vi "Run Storage Tests.vi"(8 "error in (no error)":errorcluster, 11 "Work Folder":path) -> (0 "error out":errorcluster, 2 "Report":string, 3 "All Passed":bool)   [LabVIEW 2026]
doc: "Runs every Storage test VI (Tests\\Storage) and reports one overall result. Test Data Folder is Tests\\Storage\\Test Data next to this VI; each test copies what it needs from there into a new case folder under Work Folder, so the tests can be repeated and never touch the real data in %LOCALAPPDATA%\\LVTimeTracker. An empty Work Folder (or Not a Path) means the system temp folder, in a subfolder named LVTimeTracker Tests.\n\nAll Passed is TRUE only when every test passed; Report holds every check of every test.\n\nGenerated by: Claude"
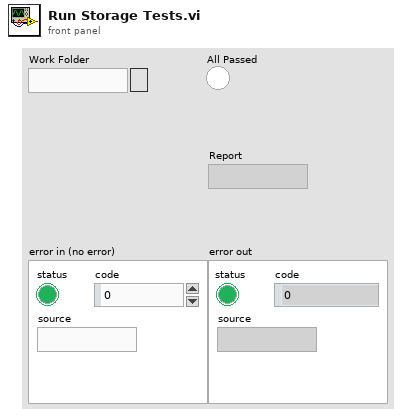
[diagram p1: front panel]
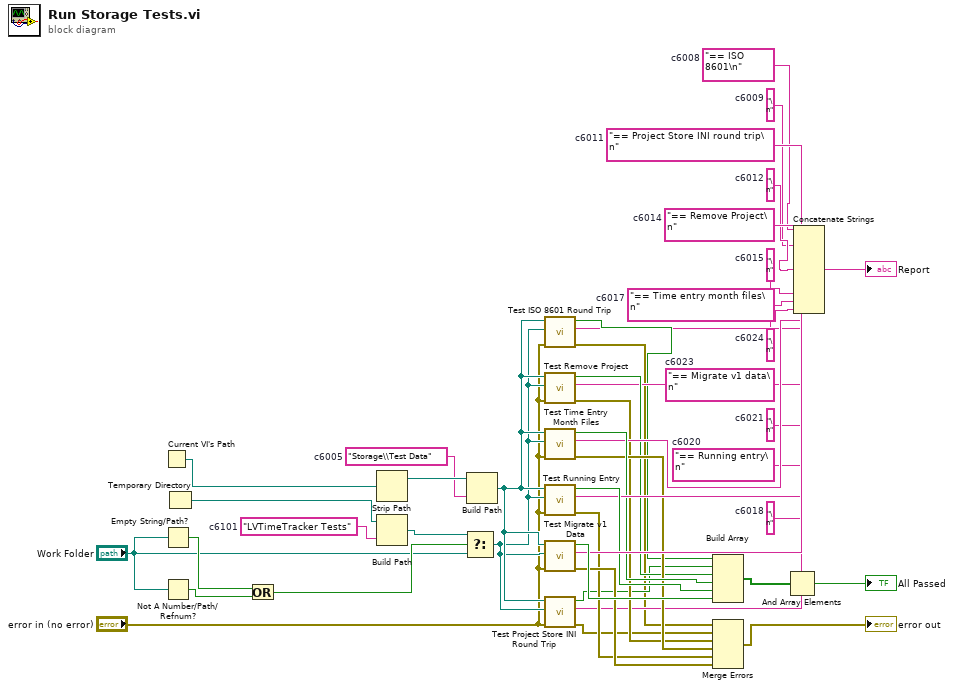
[diagram p0: block diagram]
diagram:
  w20 = "LVTimeTracker Tests"  # c6101
  w18 = "\n"  # c6024
  w17 = "== Migrate v1 data\n"  # c6023
  w16 = "\n"  # c6021
  w15 = "== Running entry\n"  # c6020
  w14 = "\n"  # c6018
  w13 = "== Time entry month files\n"  # c6017
  w12 = "\n"  # c6015
  w11 = "== Remove Project\n"  # c6014
  w10 = "\n"  # c6012
  w9 = "== Project Store INI round trip\n"  # c6011
  w8 = "\n"  # c6009
  w7 = "== ISO 8601\n"  # c6008
  w6 = "Storage\\Test Data"  # c6005
  n1 = Current VI's Path() -> (path=w26:path)
  n2 = Empty String/Path?(string/path="Work Folder") -> (empty?=w22:bool)
  n3 = Not A Number/Path/Refnum?(number/path/refnum="Work Folder") -> (NaN/Path/Refnum?=w23:bool)
  n4 = Temporary Directory() -> (w19:path)
  n5 = Or(x=w22, y=w23) -> (x .or. y?=w24:bool)
  n6 = Strip Path(path=w26) -> (stripped path=w27:path)  [unwired: 1 out]
  n7 = Build Path(base path=w19, name or relative path=w20) -> (appended path=w21:path)
  n8 = Select(t=w21, s=w24, f="Work Folder") -> (s? t:f=w25:path)
  n9 = Build Path(base path=w27, name or relative path=w6) -> (appended path=w28:path)
  n10 = call "Test ISO 8601 Round Trip.vi"("error in (no error)"="error in (no error)", "Work Folder"=w25, "Test Data Folder"=w28) -> ("error out"=w29:errorcluster, "Report"=w30:string, "Passed"=w31:bool)  [unwired: 6 in]
  n11 = call "Test Remove Project.vi"("error in (no error)"="error in (no error)", "Work Folder"=w25, "Test Data Folder"=w28) -> ("error out"=w35:errorcluster, "Report"=w36:string, "Passed"=w37:bool)  [unwired: 6 in]
  n12 = call "Test Time Entry Month Files.vi"("error in (no error)"="error in (no error)", "Work Folder"=w25, "Test Data Folder"=w28) -> ("error out"=w38:errorcluster, "Report"=w39:string, "Passed"=w40:bool)  [unwired: 6 in]
  n13 = call "Test Running Entry.vi"("error in (no error)"="error in (no error)", "Work Folder"=w25, "Test Data Folder"=w28) -> ("error out"=w41:errorcluster, "Report"=w42:string, "Passed"=w43:bool)  [unwired: 6 in]
  n14 = call "Test Migrate v1 Data.vi"("error in (no error)"="error in (no error)", "Work Folder"=w25, "Test Data Folder"=w28) -> ("error out"=w44:errorcluster, "Report"=w45:string, "Passed"=w46:bool)  [unwired: 6 in]
  n15 = call "Test Project Store INI Round Trip.vi"("error in (no error)"="error in (no error)", "Work Folder"=w25, "Test Data Folder"=w28) -> ("error out"=w32:errorcluster, "Report"=w33:string, "Passed"=w34:bool)  [unwired: 6 in]
  n16 = Build Array(w31, w34, w37, w40, w43, w46) -> (w47:bool[])
  n17 = Merge Errors(w29, w32, w35, w38, w41, w44) -> (→"error out":errorcluster)
  n18 = And Array Elements(Boolean array=w47) -> (logical AND=→"All Passed":bool)
  n19 = Concatenate Strings(w7, w30, w8, w9, w33, w10, w11, w36, w12, w13, w39, w14, w15, w42, w16, w17, w45, w18) -> (→"Report":string)
